vi "Handle Command.vi"(8 "error in (no error)":errorcluster, 9 "Value":bool, 11 "SequencedValves in":refnum<class "TriggerDelayControl.lvclass">) -> (0 "error out":errorcluster, 3 "SequencedValves out":refnum<class "TriggerDelayControl.lvclass">)   [LabVIEW 2020, in "VolatusControl.lvlib" / "TriggerDelayControl.lvclass"]
uses:
  TriggerDelayControl.lvclass
  TriggerDelayControl.lvclass/TriggerDelayControl.ctl
  State.ctl
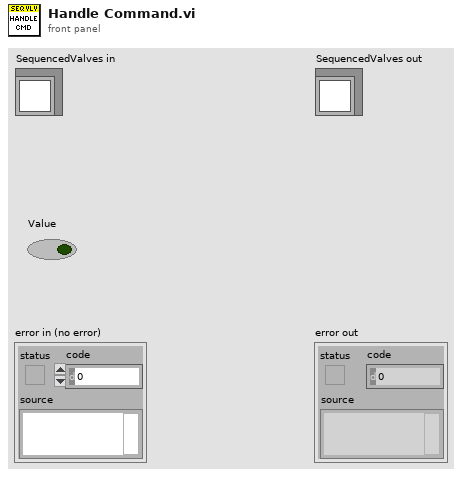
[diagram p1: front panel]
types:
  T1 = typedef "VolatusControl.lvlib/TriggerDelayControl.lvclass/State.ctl" = enum16{"Idle", "Start", "Trigger", "Delay"}
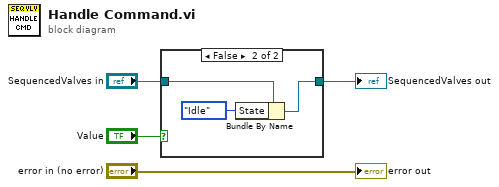
[diagram p0: block diagram]
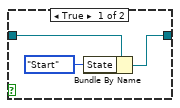
[diagram p2: hidden frame]
diagram:
  n1 = case shown="False" "Value" {
    tunnel: "SequencedValves in" -> [w7 w10]
    tunnel: [w5 w8] -> w2
    frame True {
      n2 = Bundle By Name(cluster=w7, "State"=State."Start") -> (w5:refnum<class "TriggerDelayControl.lvclass">)
    }
    frame False {
      n3 = Bundle By Name(cluster=w10, "State"=State."Idle") -> (w8:refnum<class "TriggerDelayControl.lvclass">)
    }
  }
  "SequencedValves out" <- w2
  "error out" <- "error in (no error)"
